vi "wiringPiSetupGpio.vi"(8 "error in (no error)":errorcluster) -> (0 "error out":errorcluster, 3 "status":i32)   [LabVIEW 2020, in "wiringPi.lvlib"]
doc: "<b>_______________________________________________________________</b>\n** Author: Juan José Villacorta\n** LabVIEW wrapper for C library <b> wiringPi </b>,\n** https://github.com/WiringPi/WiringPi\n<b>_______________________________________________________________</b>\n\n\n/*\n * wiringPiSetupGpio:\n * Must be called once at the start of your program execution.\n *\n * GPIO setup: Initialises the system into GPIO Pin mode and uses the\n * memory mapped hardware directly.\n *********************************************************************************\n */"
uses:
  wiringPi.lvlib
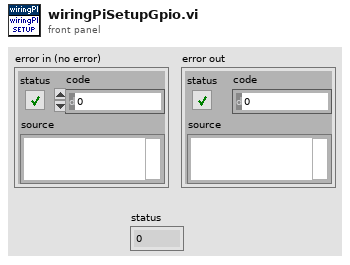
[diagram p1: front panel]
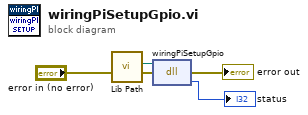
[diagram p0: block diagram]
diagram:
  n1 = call "Lib Path.vi"() -> ("path out"=w2:path)  [unwired: 11 in]
  n2 = dll-call lib="libLVwiringPi.so" fn="wiringPiSetupGpio"(path in=w2, error in="error in (no error)") -> (error out=→"error out":errorcluster, "status"=→"status":i32)  [unwired: 1 in, 1 out]
